vi "Emergancy Switch .vi"(8 "error in":errorcluster) -> (0 "error out":errorcluster, 2 "Result":string, 3 "Pressed":bool)   [LabVIEW 2021]
uses:
  DUT/DUT_Cmd.ctl
panel:
  out "Result":bool
  out "number 2":dbl
  out "Command Response 2":string
  out "Pressed 2":bool
  out "number":dbl
  out "Command Response":string
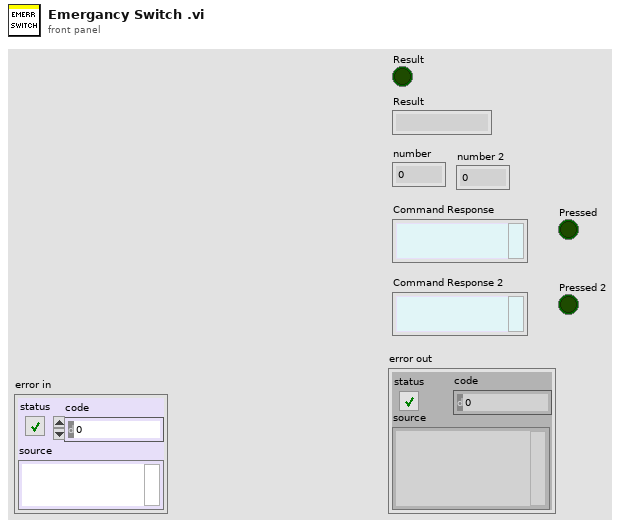
[diagram p1: front panel]
types:
  T1 = typedef "DUT_Cmd.ctl" = enum16{"Unlock serial", "Stop console logs", "Release emergency at start", "Read firmware", "WiFi credentials", "WiFi connected", "WiFi SSID", "Board revision", "ADC_NTC_TEMP", "ADC_TYPE2_RCD_CURRENT", "PCBA serial write", "PCBA serial readback", "Start energy meter", "Energy meter Vac", "Energy meter Iac", "Energy meter PF", "Energy meter energy", "Provision", "Set gateway identity", "CP checklist", "Earth detect", "D+M sense unplugged", "D+M sense plugged", "Output relay weld", "Start diagnostics", "Relay 1 on", "Relay 2 on", "Emergency pressed", "Release emergency", "Emergency released", "Unlock serial for 5 A", "Board current (5 A)", "Unlock serial for 15 A", "Board current (15 A)", "Unlock serial for 0 A", "NFC tag", "Start diagnostics again", "Relay 2 off", "Relay 1 off", "End diagnostics", "Load current (5 A) [No USB station]", "Load current (15 A) [No USB station]", "Load current (0 A) [No USB station]", "NFC tag [No USB station]", "Battery Voltage", "FW Power reset", "Notification LED", "O/P Relay weld Detection", "Earth Detection", "12V ", "5V", "3.3V"}
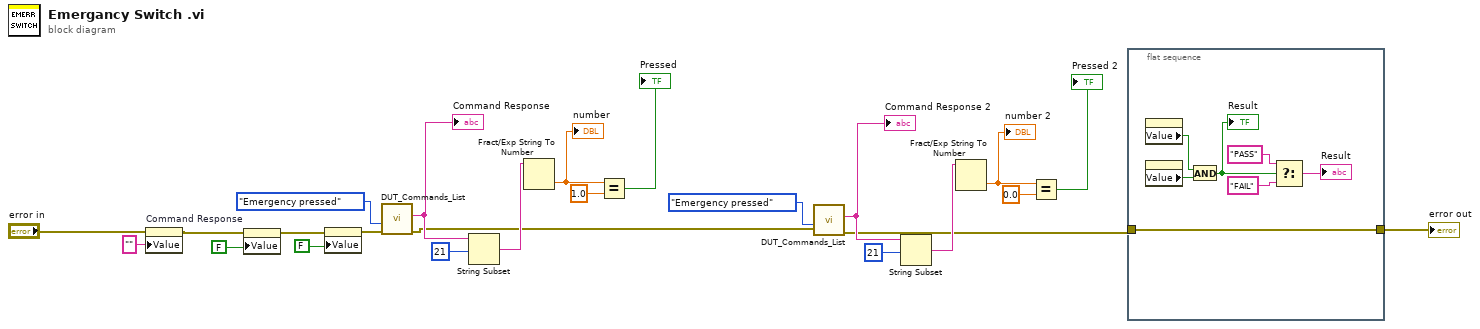
[diagram p0: block diagram]
diagram:
  n1 = property on="Command Response" class="Str"(error in="error in", "Value"="" ("Command Response")) -> (error out=w4:errorcluster)  [unwired: 1 in, 1 out]
  n2 = property on="Pressed" class="Bool (strict)"(error in=w4, "Value"=FALSE ("Pressed")) -> (error out=w5:errorcluster)  [unwired: 1 in, 1 out]
  n3 = property on="Pressed 2" class="Bool (strict)"(error in=w5, "Value"=FALSE ("Pressed 2")) -> (error out=w3:errorcluster)  [unwired: 1 in, 1 out]
  n4 = call "DUT_Commands_List.vi"("error in"=w3, "DUT Cmd"=DUT_Cmd."Emergency pressed") -> ("error out"=w8:errorcluster, "Command Response"=w21:string)  [unwired: 7 in, 1 out]
  "Command Response" <- w21
  n5 = String Subset(string=w21, offset (0)=21) -> (substring=w19:string)  [unwired: 1 in]
  n6 = Fract/Exp String To Number(string=w19) -> (number=w18:dbl)  [unwired: 3 in, 1 out]
  "number" <- w18
  n7 = Equal?(x=w18, y=1.0) -> (x = y?=→"Pressed":bool)
  n8 = call "DUT_Commands_List.vi"("error in"=w8, "DUT Cmd"=DUT_Cmd."Emergency pressed") -> ("error out"=w7:errorcluster, "Command Response"=w14:string)  [unwired: 7 in, 1 out]
  "Command Response 2" <- w14
  n9 = String Subset(string=w14, offset (0)=21) -> (substring=w12:string)  [unwired: 1 in]
  n10 = Fract/Exp String To Number(string=w12) -> (number=w11:dbl)  [unwired: 3 in, 1 out]
  "number 2" <- w11
  n11 = Equal?(x=w11, y=0.0) -> (x = y?=→"Pressed 2":bool)
  n12 = flat-sequence {
    tunnel: w7 -> [w25]
    tunnel: [w25] -> w6
    frame #0 {
      n13 = property on="Pressed" class="Bool (strict)"() -> ("Value"=w29:bool)  [unwired: 2 in, 2 out]
      n14 = property on="Pressed 2" class="Bool (strict)"() -> ("Value"=w30:bool)  [unwired: 2 in, 2 out]
      n15 = And(x=w29, y=w30) -> (x .and. y?=w31:bool)
      "Result" <- w31
      n16 = Select(t="PASS", s=w31, f="FAIL") -> (s? t:f=→"Result":string)
    }
  }
  "error out" <- w6
